vi "Move.vi"(6 "Speed (0-30)":dbl=20.0, 9 "Distance (mm)":i32=2880) -> ()   [LabVIEW 2017]
uses:
  <vilib>/FPGAPlugInAG/myRIO-1900/niLvFpga_Open_myRIO-1900.vi
  <vilib>/rvi/interface/common/dynamic/niFpgaDynamicAddResources.vi
  <vilib>/Utility/error.llb/Error Cluster From Error Code.vi
  <vilib>/rvi/errors/niLvFpgaAdjustHostInterfaceError.vi
  <vilib>/FPGAPlugInAG/Dynamic/niLvFpga_Run_Dynamic.vi
  <vilib>/FPGAPlugInAG/Dynamic/niLvFpga_Close_Dynamic.vi
  <vilib>/rvi/interface/nirviOpenFPGA/nirviOpenFPGA.xnode
  FPGA Bitfiles/BadassLoader_FPGATarget_DCMotorControlle_4dRX-8eX8o0.lvbitx
  <vilib>/rvi/interface/nirviReadWriteControl/nirviReadWriteControl.xnode
  <vilib>/rvi/interface/nirviMethod/nirviMethod.xnode
  <vilib>/rvi/interface/nirviCloseFPGA/nirviCloseFPGA.xnode
  NiFpgaLv.dll
  <vilib>/rvi/interface/Simulation/niFpgaSimulationCallBeginRW.vi
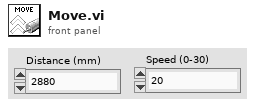
[diagram p1: front panel]
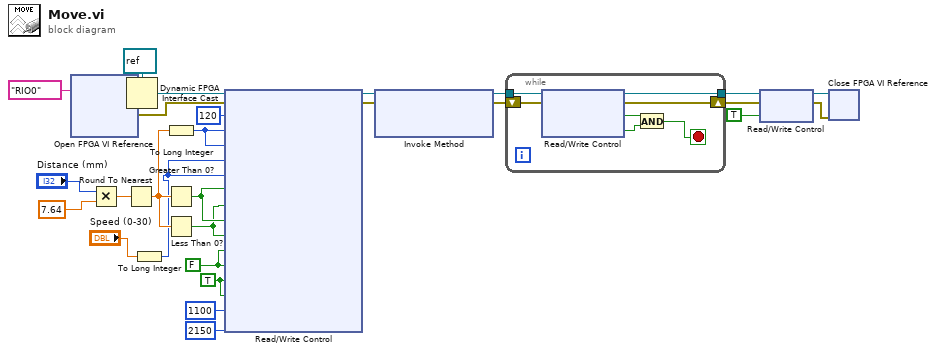
[diagram p0: block diagram]
diagram:
  w3 = TRUE ("S 5")
  w4 = FALSE ("stop")
  n1 = xnode "Open FPGA VI Reference"("resource name"=tag "RIO0") -> ("FPGA VI Reference Out"=w22:refnum<k20>, "error out"=w20:errorcluster)  [unwired: 1 in]
  n2 = Multiply(x="Distance (mm)", y=7.64) -> (x*y=w24:dbl)
  n3 = Round To Nearest(number=w24) -> (nearest integer value=w9:dbl)
  n4 = Dynamic FPGA Interface Cast(Session In=refnum<k20> refnum ("FPGA Interface"), Type=w22) -> (Session Out=w21:refnum<k20>)
  n5 = To Long Integer(number="Speed (0-30)") -> (32bit integer=w5:i32)
  n6 = To Long Integer(number=w9) -> (32bit integer=w19:i32)
  n7 = Greater Than 0?(x=w9) -> (x > 0?=w10:bool)
  n8 = Less Than 0?(x=w9) -> (x < 0?=w8:bool)
  n9 = xnode "Read/Write Control"("FPGA VI Reference In"=w21, "error in"=w20, "Ticks to slow"=120, "DCmotor_0_enc trgt"=w19, "DCmotor_1_enc trgt"=w19, "DCmotor_0_ccw vel sp"=w5, "DCmotor_1_ccw vel sp"=w5, "DCmotor_0_A"=w10, "DCmotor_0_B"=w8, "DCmotor_1_A"=w10, "DCmotor_1_B"=w8, "invert pulse (F)"=w4, "stop"=w4, "S 5"=w3, "S 6"=w3, "Servo 5"=u32 1100, "Servo 6"=u32 2150) -> ("FPGA VI Reference Out"=w16:refnum<k20>, "error out"=w15:errorcluster)
  n10 = xnode "Invoke Method"("FPGA VI Reference In"=w16, "error in"=w15) -> ("FPGA VI Reference Out"=w14:refnum<k20>, "error out"=w13:errorcluster)  [unwired: 1 in]
  n11 = while {
    tunnel: w14 -> [w35]
    tunnel: [w32] -> w18
    shift-right: [w30] -> w12
    shift-left: w13 -> [w31]
    stop <- w29 stop-if-true
    n12 = xnode "Read/Write Control"("FPGA VI Reference In"=w35, "error in"=w31) -> ("FPGA VI Reference Out"=w32:refnum<k20>, "error out"=w30:errorcluster, "M0_finished"=w34:bool, "M1_finished"=w33:bool)
    n13 = And(x=w34, y=w33) -> (x .and. y?=w29:bool)
  }
  n14 = xnode "Read/Write Control"("FPGA VI Reference In"=w18, "error in"=w12, "stop"=TRUE) -> ("FPGA VI Reference Out"=w28:refnum<k20>, "error out"=w27:errorcluster)
  n15 = xnode "Close FPGA VI Reference"("FPGA VI Reference In"=w28, "error in"=w27) -> ()  [unwired: 1 out]
